vi "Host_main_Lab9.vi"() -> ()   [LabVIEW 2025]
uses:
  vi/thresholds.ctl
  UI_Msg.ctl
  action.ctl
  states.ctl
panel:
  in  "Files":i32(listbox)
  in  "local folder path":path
  in  "user":string
  in  "password":string
  out "cmd_ok":bool
  in  "Stop RT":bool
  out "Connected?":bool
  in  "IP myRIO":string="172.22.11.2"
  out "error out":errorcluster
  in  "Manual trigger":bool
  in  "parameters":T1
  out "Waveform Graph":i16[][](graph)
  in  "Close":bool
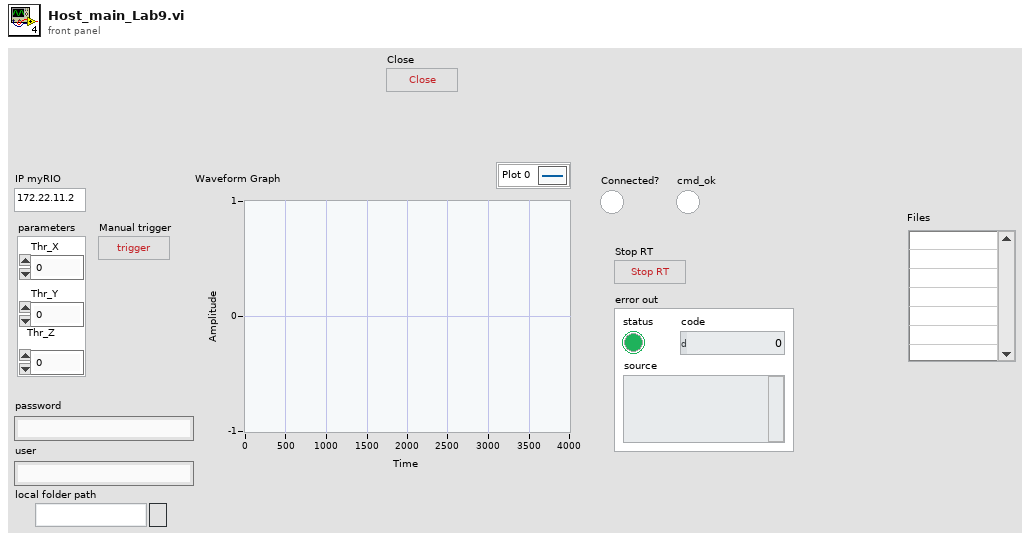
[diagram p1: front panel]
types:
  T1 = typedef "thresholds.ctl" = cluster{"Thr_X":i16, "Thr_Y":i16, "Thr_Z":i16}
  T2 = enum32{"invalid app kind", "Development System", "Run Time System", "Student Edition", "Embedded LabVIEW", "Evaluation", "Custom"}
  T3 = typedef "states.ctl" = enum16{"Run", "Connect"}
  T4 = typedef "UI_Msg.ctl" = cluster{"action":T5, "Threshold":T1, "file name":string}
  T5 = typedef "action.ctl" = enum16{"Thresholds_Changed", "Manual_Trigger", "Stop", "remove_file"}
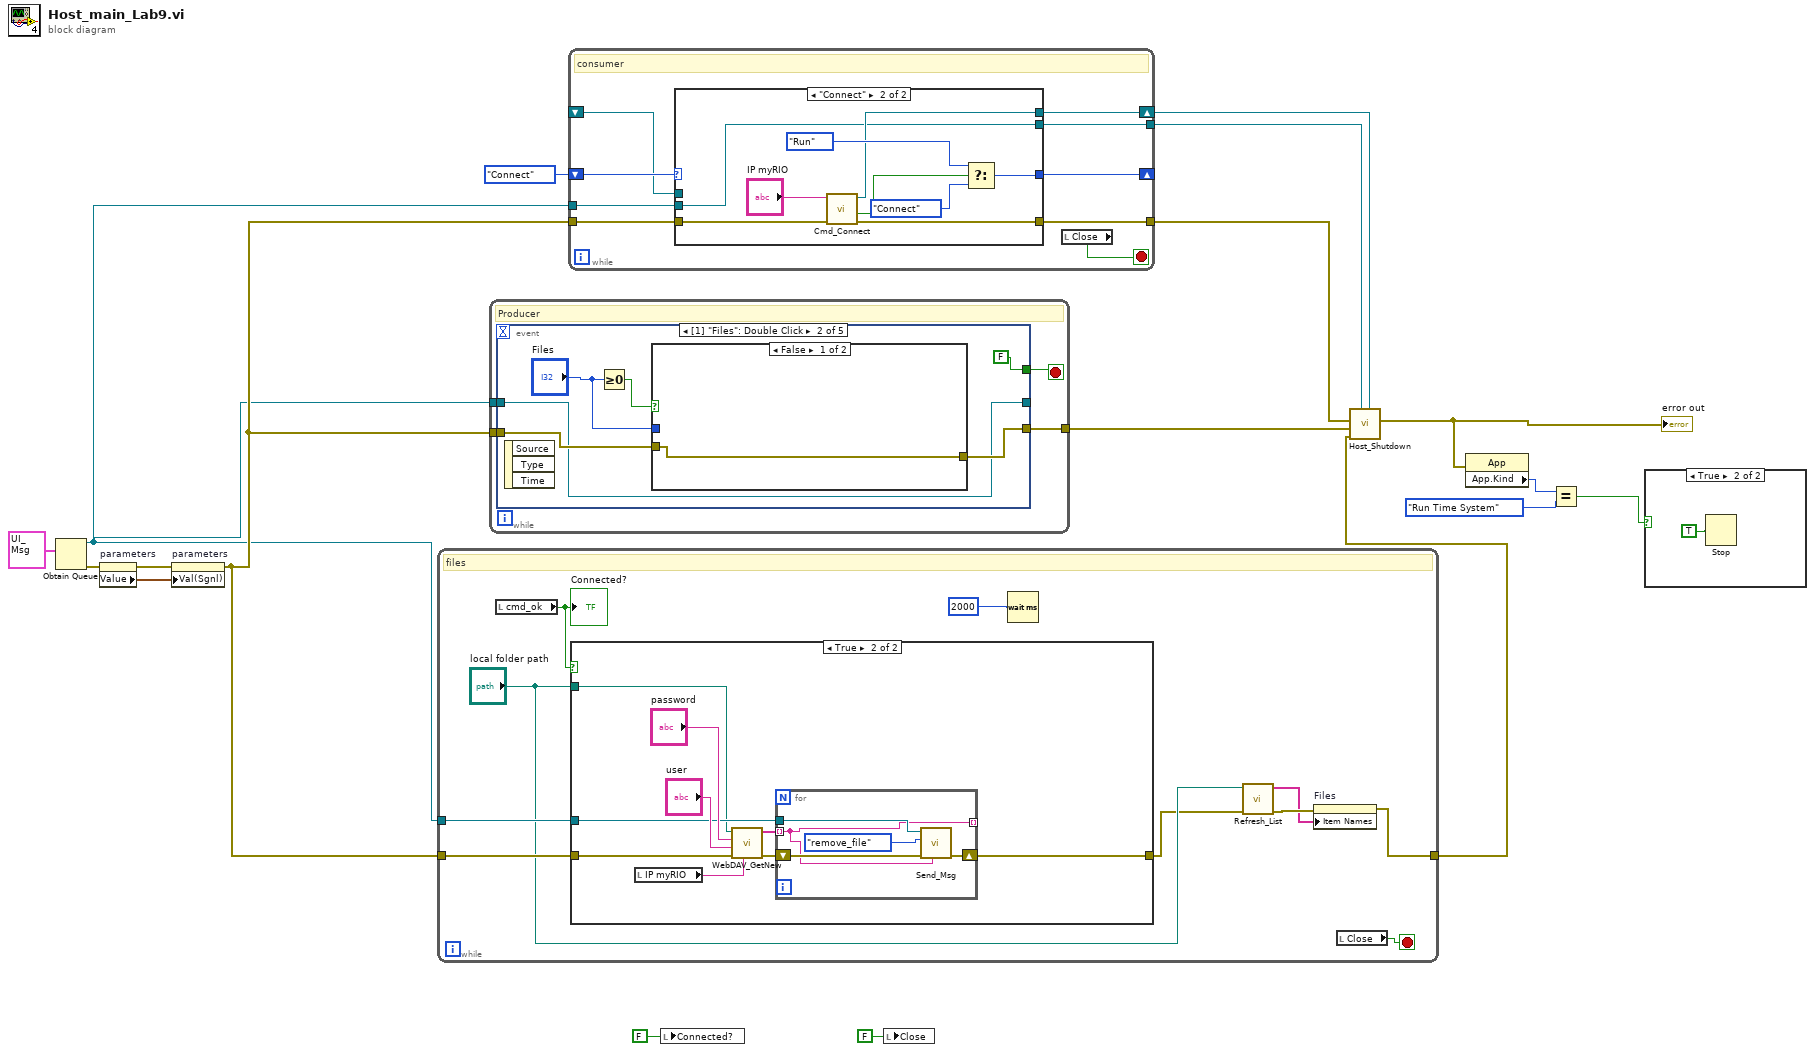
[diagram p0: block diagram]
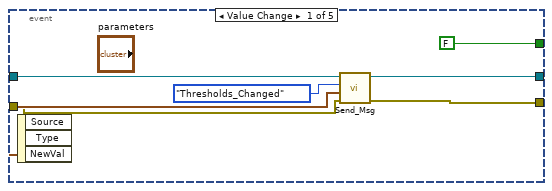
[diagram p3: hidden frame]
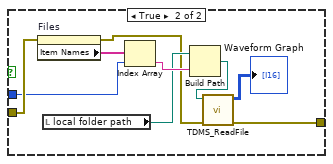
[diagram p4: hidden frame]
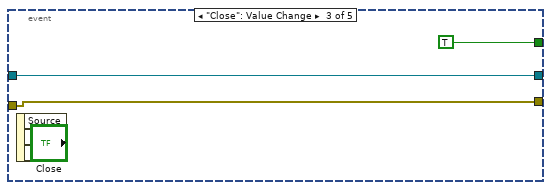
[diagram p5: hidden frame]
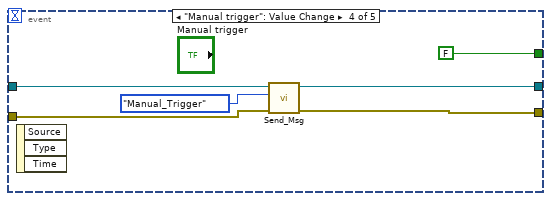
[diagram p6: hidden frame]
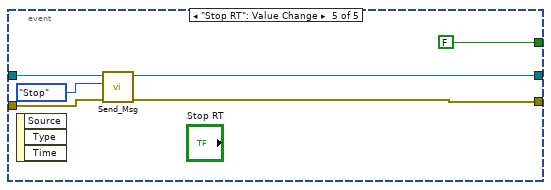
[diagram p7: hidden frame]
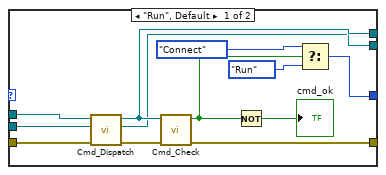
[diagram p8: hidden frame]
diagram:
  n1 = Obtain Queue(element data type=T4 {"action"=enum."Thresholds_Changed", "Threshold"={"Thr_X"=0, "Thr_Y"=0, "Thr_Z"=0}, "file name"=""} ("msg")) -> (queue out=w5:refnum<queue>, error out=w13:errorcluster)  [unwired: 4 in, 1 out]
  n2 = property on="parameters" class="Clust (strict)"(error in=w13) -> (error out=w17:errorcluster, "Value"=w16:T1)  [unwired: 1 in, 1 out]
  n3 = property on="parameters" class="Clust (strict)"(error in=w17, "Val(Sgnl)"=w16) -> (error out=w7:errorcluster)  [unwired: 1 in, 1 out]
  n4 = while {
    tunnel: w7 -> [w25]
    tunnel: [w20] -> w6
    tunnel: w5 -> [w26]
    stop <- w28 stop-if-true
    # "files"
    n5 = local read "cmd_ok"() -> (w27:bool)
    "Connected?" <- w27
    n6 = case shown="True" w27 {
      tunnel: w26 -> [_ w32]
      tunnel: w25 -> [_ w34]
      tunnel: "local folder path" -> [_ w30]
      tunnel: [_ w29] -> w22
      frame False {
      }
      frame True {
        n7 = local read "IP myRIO"() -> (w37:string)
        n8 = call "WebDAV_GetNew.vi"("IP myRIO"=w37, "error in (no error)"=w34, "user"="user", "password"="password", "local file path"=w30) -> ("error out"=w33:errorcluster, "dowloads"=w31:string[])  [unwired: 5 in]
        n9 = for {
          shift-right: [w40] -> w29
          shift-left: w33 -> [w41]
          tunnel: w32 -> [w42]
          tunnel: [w39] -> _ mode=indexing
          tunnel: w31 -> [w39] mode=indexing
          n10 = call "Send_Msg.vi"("file name"=w39, "error in (no error)"=w41, "action"=action."remove_file", "Queue in"=w42) -> ("error out"=w40:errorcluster)  [unwired: 6 in, 1 out]
        }
      }
    }
    n11 = Wait (ms)(milliseconds to wait=u32 2000) -> ()  [unwired: 1 out]
    n12 = call "Refresh_List.vi"("error in (no error)"=w22, "path"="local folder path") -> ("error out"=w21:errorcluster, "reversed array"=w19:string[])  [unwired: 8 in]
    n13 = property on="Files" class="LstBox (strict)"(error in=w21, "Item Names"=w19) -> (error out=w20:errorcluster)  [unwired: 1 in, 1 out]
    n14 = local read "Close"() -> (w28:bool)
  }
  n15 = while {
    tunnel: w7 -> [w45]
    tunnel: w5 -> [w43]
    tunnel: [w44] -> w8
    stop <- w46 stop-if-true
    # "Producer"
    n16 = event shown="[1] \"Files\": Double Click" {
      selector: _ -> [_ _ _ _ _]
      dyn-events: _ -> [_ _ _ _ _]
      timeout: _ -> [_ _ _ _ _]
      tunnel: [FALSE FALSE TRUE FALSE FALSE] -> w46
      tunnel: [w50 w54 w71 w75 w79] -> _
      tunnel: w45 -> [w49 w57 w70 w78 w81]
      tunnel: [w48 w56 w70 w74 w80] -> w44
      tunnel: w43 -> [w51 w54 w71 w77 w82]
      event Value Change {
        n17 = event-data() -> ("NewVal"=w52:T1)  [unwired: 1 in, 2 out]
        n18 = call "Send_Msg.vi"("error in (no error)"=w49, "NewVal"=w52, "action"=action."Thresholds_Changed", "Queue in"=w51) -> ("error out"=w48:errorcluster, "Queue out"=w50:refnum<queue>)  [unwired: 6 in]
      }
      event "Files": Double Click {
        n19 = event-data() -> ()  [unwired: 1 in, 3 out]
        n20 = Greater Or Equal To 0?(x="Files") -> (x >= 0?=w59:bool)
        n21 = case shown="False" w59 {
          tunnel: "Files" -> [_ w67]
          tunnel: w57 -> [w60 w69]
          tunnel: [w60 w62] -> w56
          frame False {
          }
          frame True {
            n22 = property on="Files" class="LstBox (strict)"(error in=w69) -> (error out=w63:errorcluster, "Item Names"=w68:string[])  [unwired: 1 in, 1 out]
            n23 = local read "local folder path"() -> (w65:path)
            n24 = Index Array(array=w68, index=w67) -> (element=w66:string)
            n25 = Build Path(base path=w65, name or relative path=w66) -> (appended path=w64:path)
            n26 = call "TDMS_ReadFile.vi"("error in (no error)"=w63, "file path"=w64) -> ("error out"=w62:errorcluster, "data"=→"Waveform Graph":i16[][])  [unwired: 8 in]
          }
        }
      }
      event "Close": Value Change {
        n27 = event-data() -> ()  [unwired: 1 in, 3 out]
      }
      event "Manual trigger": Value Change {
        n28 = event-data() -> ()  [unwired: 1 in, 3 out]
        n29 = call "Send_Msg.vi"("error in (no error)"=w78, "action"=action."Manual_Trigger", "Queue in"=w77) -> ("error out"=w74:errorcluster, "Queue out"=w75:refnum<queue>)  [unwired: 7 in]
      }
      event "Stop RT": Value Change {
        n30 = event-data() -> ()  [unwired: 1 in, 3 out]
        n31 = call "Send_Msg.vi"("error in (no error)"=w81, "action"=action."Stop", "Queue in"=w82) -> ("error out"=w80:errorcluster, "Queue out"=w79:refnum<queue>)  [unwired: 7 in]
      }
    }
  }
  n32 = while {
    shift-right: [w91] -> _
    shift-left: states."Connect" ("Enum") -> [w93]
    tunnel: w7 -> [w92]
    shift-right: [w90] -> w10
    shift-left: _ -> [w89]
    tunnel: w5 -> [w88]
    tunnel: [w86] -> w11
    tunnel: [w85] -> w9
    stop <- w87 stop-if-true
    # "consumer"
    n33 = case shown="\"Connect\"" w93 {
      tunnel: [w97 w109] -> w85
      tunnel: w92 -> [w103 w111]
      tunnel: [w99 w112] -> w91
      tunnel: [w98 w107] -> w90
      tunnel: w89 -> [w105 _]
      tunnel: w88 -> [w104 w106]
      tunnel: [w94 w106] -> w86
      frame "Run", Default {
        n34 = call "Cmd_Dispatch.vi"("error in"=w103, "queue in"=w104, "writer endpoint in"=w105) -> ("error Iout"=w102:errorcluster, "queue out"=w94:refnum<queue>, "writer endpoint out"=w98:refnum<k21>)  [unwired: 6 in]
        n35 = call "Cmd_Check.vi"("error in"=w102, "writer ref in"=w98) -> ("error out"=w97:errorcluster, "disconnected?"=w96:bool)  [unwired: 8 in]
        n36 = Not(x=w96) -> (.not. x?=→"cmd_ok":bool)
        n37 = Select(t=states."Connect" ("Enum"), s=w96, f=states."Run" ("Enum")) -> (s? t:f=w99:T3)
      }
      frame "Connect" {
        n38 = call "Cmd_Connect.vi"("error in (no error)"=w111, "IP myRIO in"="IP myRIO") -> ("error out"=w109:errorcluster, "connected?"=w108:bool, "Refnum out"=w107:refnum<k21>)  [unwired: 7 in]
        n39 = Select(t=states."Run" ("Enum"), s=w108, f=states."Connect") -> (s? t:f=w112:T3)
      }
    }
    n40 = local read "Close"() -> (w87:bool)
  }
  n41 = local write "Connected?"(FALSE ("Connected?")) -> ()
  n42 = local write "Close"(FALSE ("Stop")) -> ()
  n43 = call "Host_Shutdown.vi"("writer ref"=w10, "Queue in"=w11, "error in 2"=w6, "error in 1"=w8, "error in 3"=w9) -> ("error out"=w4:errorcluster)  [unwired: 6 in]
  "error out" <- w4
  n44 = property class="App"(error in=w4) -> ("App.Kind"=w3:T2)  [unwired: 1 in, 2 out]
  n45 = Equal?(x=w3, y=T2."Run Time System") -> (x = y?=w1:bool)
  n46 = case shown="True" w1 {
    frame False {
    }
    frame True {
      n47 = Stop(stop? (T)=TRUE) -> ()
    }
  }
